vi "VM - Get list of contexts.vi"(6 "error in":errorcluster, 9 "Creator (all contexts)":string) -> (0 "error out":errorcluster, 1 "err code":T1 items=["No error", "Invalid variable type", "Variable not found", "Variable already exists", "Invalid context handle", "Input error", "Invalid data format", "No history attached", "History already attached", "Invalid history parameters", "Wrong variable name", "Wrong alias name", "Non-unique alias", "Alias not found", "No alias associated", "Alias already associated", "Wrong context name", "Non-unique context name", "Context name not found", "Invalid parameter", "Generic error", "Memory Full", "Unrecognized LV error", "Unknown error code"], 3 "array of VC handles":T2[](array[typedef]))   [LabVIEW 2021]
doc: "This VI returns the VC Handles of either all open contexts or contexts belonging to the specified creator. Refer to the VI help for more details.\n\nIf the <b>Creator</b> control is unwired or contains an empty string, the VI returns the handles of all local contexts. Otherwise, the VI returns the handles of the contexts that belong to <b>Creator</b>. The name of the context's creator is specified when the context is created.\n\n::: CalcExpress Toolkit :::\nCopyright (c) 2000-2026 Konstantin Shifershteyn. All rights reserved."
uses:
  cetypes.llb/VarMan Variable Context Handle.ctl
  cetypes.llb/VarMan Error Code.ctl
  cersrc/celveng32.dll
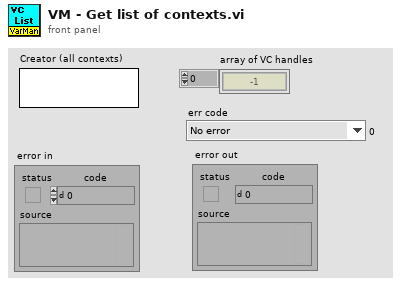
[diagram p1: front panel]
types:
  T1 = typedef "VarMan Error Code.ctl" = u16
  T2 = typedef "VarMan Variable Context Handle.ctl" = i32
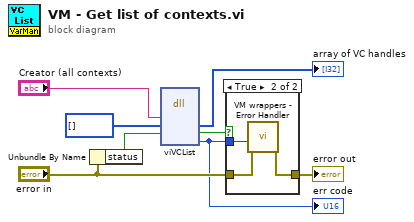
[diagram p0: block diagram]
diagram:
  n1 = Unbundle By Name("error in") -> ("status"=w4:bool)
  n2 = dll-call lib="C:/LV Projects/CalcExpress 40 LV2021/vi.lib/addons/CalcExpress/cersrc/celveng*.dll" fn="viVCList"("creator"="Creator (all contexts)", "vchArrHdl"=T2[] [] ("array of VC handles"), "errf"=w4) -> ("vchArrHdl"=→"array of VC handles":T2[], "errf"=w5:bool, "err code"=w6:T1)  [unwired: 6 in, 2 out]
  "err code" <- w6
  n3 = case shown="True" w5 {
    tunnel: [w9 w12] -> w8
    tunnel: "error in" -> [w9 w11]
    tunnel: w6 -> [_ w10]
    frame False {
    }
    frame True {
      n4 = call "VM wrappers - Error Handler.vi"("error before"=w11, "VarMan error"=w10) -> ("error out"=w12:errorcluster)  [unwired: 8 in, 1 out]
    }
  }
  "error out" <- w8
